vi "Adj Controls Pos.vi"(0 "Decoration Ref Array":refnum<vi>[](array[refnum]), 2 "Panel Bounds":T1, 11 "Control Ref Array":refnum<vi>[](array[refnum])) -> ()   [LabVIEW 2021]
uses:
  <vilib>/Utility/miscctls.llb/LVRectTypeDef.ctl
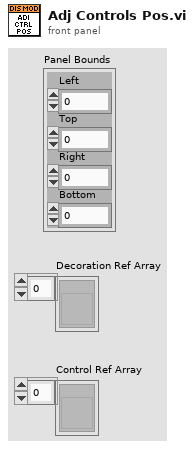
[diagram p1: front panel]
types:
  T1 = typedef "LVRectTypeDef.ctl" = cluster{"Left":i16, "Top":i16, "Right":i16, "Bottom":i16}
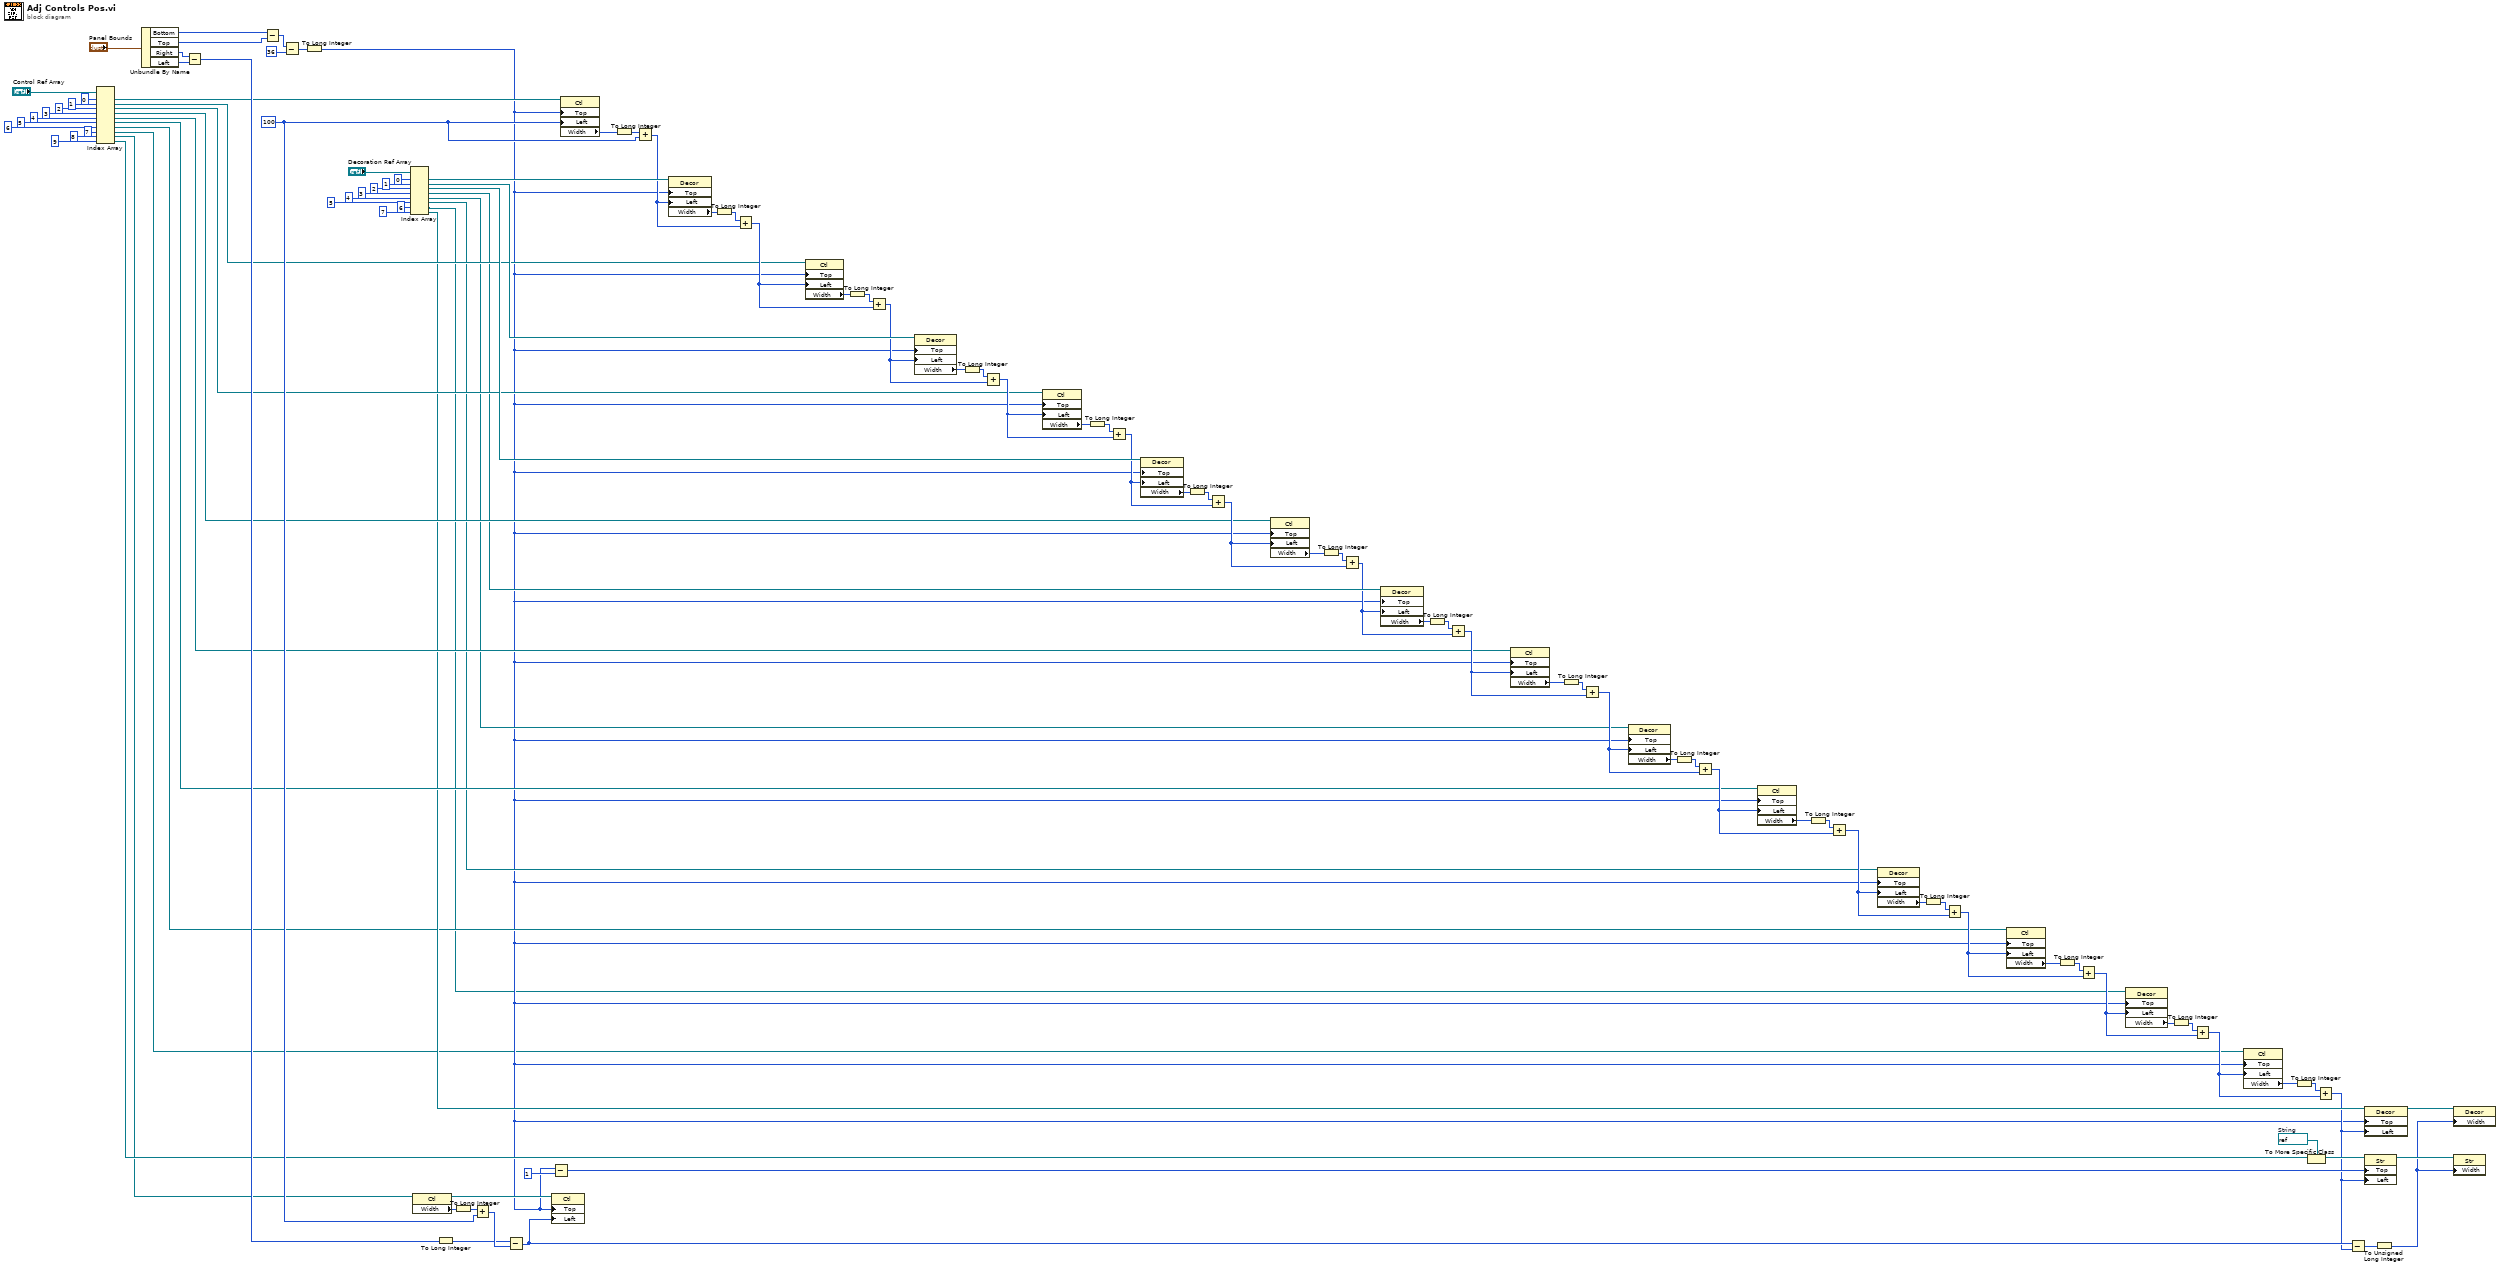
[diagram p0: block diagram]
diagram:
  w46 = refnum<vi> refnum  # String
  w100 = 100 ("Position:Left")
  n1 = Index Array(array="Control Ref Array", index #1=0 ("index"), index #2=1 ("index"), index #3=2 ("index"), index #4=3 ("index"), index #5=4 ("index"), index #6=5 ("index"), index #7=6 ("index"), index #8=7 ("index"), index #9=8 ("index"), index #10=9 ("index")) -> (element #1=w50:refnum<vi>, element #2=w49:refnum<vi>, element #3=w48:refnum<vi>, element #4=w47:refnum<vi>, element #5=w37:refnum<vi>, element #6=w26:refnum<vi>, element #7=w11:refnum<vi>, element #8=w2:refnum<vi>, element #9=w12:refnum<vi>, element #10=w13:refnum<vi>)
  n2 = Unbundle By Name("Panel Bounds") -> ("Bottom"=w105:i16, "Top"=w104:i16, "Right"=w103:i16, "Left"=w102:i16)
  n3 = Subtract(x=w103, y=w102) -> (x-y=w99:i16)
  n4 = Subtract(x=w105, y=w104) -> (x-y=w108:i16)
  n5 = Subtract(x=w108, y=i16 36) -> (x-y=w101:i16)
  n6 = To Long Integer(number=w101) -> (32bit integer=w3:i32)
  n7 = Index Array(array="Decoration Ref Array", index #1=0 ("index"), index #2=1 ("index"), index #3=2 ("index"), index #4=3 ("index"), index #5=4 ("index"), index #6=5 ("index"), index #7=6 ("index"), index #8=7 ("index")) -> (element #1=w98:refnum<vi>, element #2=w73:refnum<vi>, element #3=w67:refnum<vi>, element #4=w38:refnum<vi>, element #5=w27:refnum<vi>, element #6=w16:refnum<vi>, element #7=w1:refnum<vi>, element #8=w23:refnum<vi>)
  n8 = property class="Ctl"(reference=w12) -> (reference out=w85:refnum<vi>, "Width"=w84:u32)  [unwired: 1 in, 1 out]
  n9 = To Long Integer(number=w99) -> (32bit integer=w81:i32)
  n10 = To Long Integer(number=w84) -> (32bit integer=w83:i32)
  n11 = Add(x=w83, y=w100) -> (x+y=w82:i32)
  n12 = Subtract(x=w81, y=w82) -> (x-y=w78:i32)
  n13 = property class="Ctl"(reference=w85, "Top"=w3, "Left"=w78) -> ()  [unwired: 1 in, 2 out]
  n14 = Subtract(x=w3, y=1) -> (x-y=w95:i32)
  n15 = property class="Ctl"(reference=w50, "Top"=w3, "Left"=w100) -> ("Width"=w93:u32)  [unwired: 1 in, 2 out]
  n16 = To Long Integer(number=w93) -> (32bit integer=w92:i32)
  n17 = Add(x=w92, y=w100) -> (x+y=w87:i32)
  n18 = property class="Decor"(reference=w98, "Top"=w3, "Left"=w87) -> ("Width"=w91:u32)  [unwired: 1 in, 2 out]
  n19 = To Long Integer(number=w91) -> (32bit integer=w90:i32)
  n20 = Add(x=w90, y=w87) -> (x+y=w86:i32)
  n21 = property class="Ctl"(reference=w49, "Top"=w3, "Left"=w86) -> ("Width"=w88:u32)  [unwired: 1 in, 2 out]
  n22 = To Long Integer(number=w88) -> (32bit integer=w89:i32)
  n23 = Add(x=w89, y=w86) -> (x+y=w70:i32)
  n24 = property class="Decor"(reference=w73, "Top"=w3, "Left"=w70) -> ("Width"=w71:u32)  [unwired: 1 in, 2 out]
  n25 = To Long Integer(number=w71) -> (32bit integer=w72:i32)
  n26 = Add(x=w72, y=w70) -> (x+y=w66:i32)
  n27 = property class="Ctl"(reference=w48, "Top"=w3, "Left"=w66) -> ("Width"=w68:u32)  [unwired: 1 in, 2 out]
  n28 = To Long Integer(number=w68) -> (32bit integer=w69:i32)
  n29 = Add(x=w69, y=w66) -> (x+y=w63:i32)
  n30 = property class="Decor"(reference=w67, "Top"=w3, "Left"=w63) -> ("Width"=w64:u32)  [unwired: 1 in, 2 out]
  n31 = To Long Integer(number=w64) -> (32bit integer=w65:i32)
  n32 = Add(x=w65, y=w63) -> (x+y=w60:i32)
  n33 = property class="Ctl"(reference=w47, "Top"=w3, "Left"=w60) -> ("Width"=w61:u32)  [unwired: 1 in, 2 out]
  n34 = To Long Integer(number=w61) -> (32bit integer=w62:i32)
  n35 = Add(x=w62, y=w60) -> (x+y=w36:i32)
  n36 = property class="Decor"(reference=w38, "Top"=w3, "Left"=w36) -> ("Width"=w40:u32)  [unwired: 1 in, 2 out]
  n37 = To Long Integer(number=w40) -> (32bit integer=w39:i32)
  n38 = Add(x=w39, y=w36) -> (x+y=w43:i32)
  n39 = property class="Ctl"(reference=w37, "Top"=w3, "Left"=w43) -> ("Width"=w42:u32)  [unwired: 1 in, 2 out]
  n40 = To Long Integer(number=w42) -> (32bit integer=w41:i32)
  n41 = Add(x=w41, y=w43) -> (x+y=w28:i32)
  n42 = property class="Decor"(reference=w27, "Top"=w3, "Left"=w28) -> ("Width"=w30:u32)  [unwired: 1 in, 2 out]
  n43 = To Long Integer(number=w30) -> (32bit integer=w29:i32)
  n44 = Add(x=w29, y=w28) -> (x+y=w33:i32)
  n45 = property class="Ctl"(reference=w26, "Top"=w3, "Left"=w33) -> ("Width"=w32:u32)  [unwired: 1 in, 2 out]
  n46 = To Long Integer(number=w32) -> (32bit integer=w31:i32)
  n47 = Add(x=w31, y=w33) -> (x+y=w17:i32)
  n48 = property class="Decor"(reference=w16, "Top"=w3, "Left"=w17) -> ("Width"=w19:u32)  [unwired: 1 in, 2 out]
  n49 = To Long Integer(number=w19) -> (32bit integer=w18:i32)
  n50 = Add(x=w18, y=w17) -> (x+y=w22:i32)
  n51 = property class="Ctl"(reference=w11, "Top"=w3, "Left"=w22) -> ("Width"=w21:u32)  [unwired: 1 in, 2 out]
  n52 = To Long Integer(number=w21) -> (32bit integer=w20:i32)
  n53 = Add(x=w20, y=w22) -> (x+y=w5:i32)
  n54 = property class="Decor"(reference=w1, "Top"=w3, "Left"=w5) -> ("Width"=w7:u32)  [unwired: 1 in, 2 out]
  n55 = To Long Integer(number=w7) -> (32bit integer=w6:i32)
  n56 = Add(x=w6, y=w5) -> (x+y=w10:i32)
  n57 = property class="Ctl"(reference=w2, "Top"=w3, "Left"=w10) -> ("Width"=w9:u32)  [unwired: 1 in, 2 out]
  n58 = To Long Integer(number=w9) -> (32bit integer=w8:i32)
  n59 = To More Specific Class(target class=w46, reference=w13) -> (specific class reference=w45:refnum<vi>)  [unwired: 1 in, 1 out]
  n60 = Add(x=w8, y=w10) -> (x+y=w4:i32)
  n61 = Subtract(x=w78, y=w4) -> (x-y=w77:i32)
  n62 = property class="Decor"(reference=w23, "Top"=w3, "Left"=w4) -> (reference out=w80:refnum<vi>)  [unwired: 1 in, 1 out]
  n63 = property class="Str"(reference=w45, "Top"=w95, "Left"=w4) -> (reference out=w79:refnum<vi>)  [unwired: 1 in, 1 out]
  n64 = To Unsigned Long Integer(number=w77) -> (unsigned 32bit integer=w76:u32)
  n65 = property class="Decor"(reference=w80, "Width"=w76) -> ()  [unwired: 1 in, 2 out]
  n66 = property class="Str"(reference=w79, "Width"=w76) -> ()  [unwired: 1 in, 2 out]
